vi "read inputs from fpga.vi"(7 "FPGA ref":T6, 8 "error in":errorcluster, 9 "diagnostics":T4[](array[typedef]), 10 "inputs":T1[](array[typedef]), 11 "data table in in":T7) -> (0 "error out":errorcluster, 1 "diagnostics out":T4[](array[typedef]), 2 "inputs out":T1[](array[typedef]), 3 "data table out":T7)   [LabVIEW 2013, in "Profibus Module runtime.lvclass"]
uses:
  Profibus Module runtime.lvclass
  <vilib>/NI/Tag Bus/table/data table.ctl
  profibus diagnostics reporting.ctl
  configuration/error throw specification.ctl
  profibus slave configuration.ctl
  profibus mapping configuration.ctl
  <vilib>/NI/Tag Bus/tag/Data Type.ctl
  dynamic profibus/fpga reference.ctl
  <vilib>/NI/Tag Bus/table/data polymorphs/write one/write Array of U8.vi
  dynamic profibus/dynamic profibus.lvlib
  <vilib>/NI/Tag Bus/table/data table.lvlib
  configuration/Profibus Module configuration.lvclass
  <vilib>/NI/Tag Bus/tag/tag descriptor.lvclass
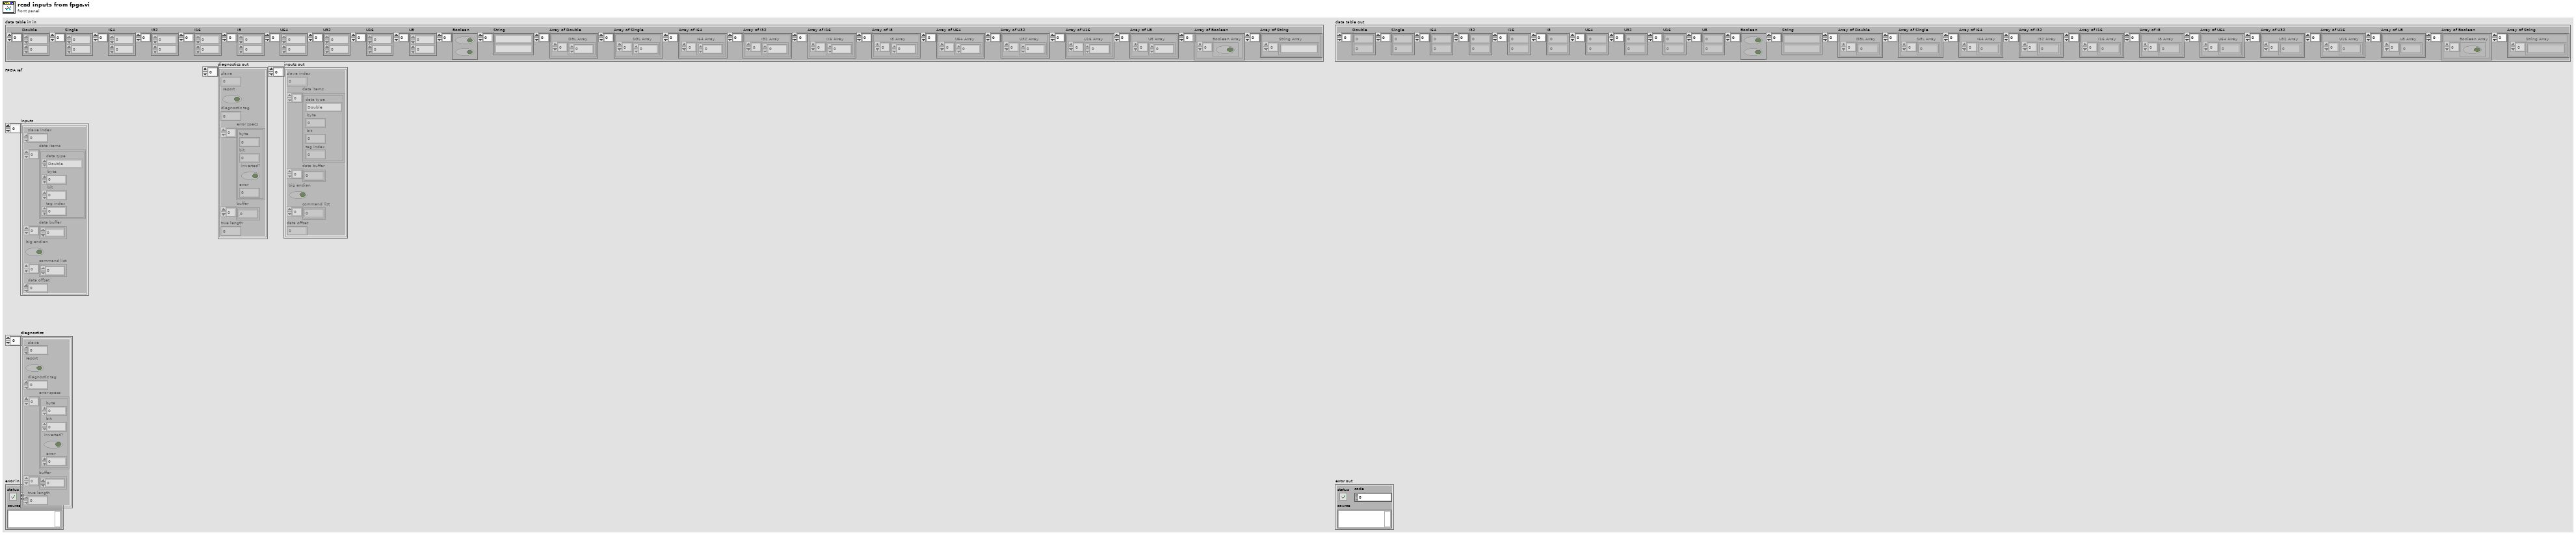
[diagram p1: front panel]
types:
  T1 = typedef "Profibus Module runtime.lvclass/profibus slave configuration.ctl" = cluster{"slave index":i8, "data items":T2[], "data buffer":u8[], "big endian":bool, "command list":u32[], "data offset":u8}
  T2 = typedef "Profibus Module runtime.lvclass/profibus mapping configuration.ctl" = cluster{"data type":T3, " byte":i32, " bit":i32, "tag index":i32}
  T3 = typedef "tag bus.lvlib/tag descriptor.lvclass/Data Type.ctl" = enum16{"Double", "Single", "I64", "I32", "I16", "I8", "U64", "U32", "U16", "U8", "Boolean", "String", "Array of Double", "Array of Single", "Array of I64", "Array of I32", "Array of I16", "Array of I8", "Array of U64", "Array of U32", "Array of U16", "Array of U8", "Array of Boolean", "Array of String"}
  T4 = typedef "Profibus Module runtime.lvclass/profibus diagnostics reporting.ctl" = cluster{"slave":i8, "report":bool, "diagnostic tag":i32, "error specs":T5[], "buffer":u8[], "true length":u8}
  T5 = typedef "Profibus Module configuration.lvclass/error throw specification.ctl" = cluster{"byte":i32, "bit":i32, "inverted?":bool, "error":i32}
  T6 = typedef "dynamic profibus.lvlib/fpga reference.ctl" = refnum<k20>
  T7 = typedef "tag bus.lvlib/data table.lvlib/data table.ctl" = cluster{"Double":dbl[], "Single":sgl[], "I64":i64[], "I32":i32[], "I16":i16[], "I8":i8[], "U64":u64[], "U32":u32[], "U16":u16[], "U8":u8[], "Boolean":bool[], "String":string[], "Array of Double":cluster{"DBL Array":dbl[]}[], "Array of Single":cluster{"SGL Array":sgl[]}[], "Array of I64":cluster{"I64 Array":i64[]}[], "Array of I32":cluster{"I32 Array":i32[]}[], "Array of I16":cluster{"I16 Array":i16[]}[], "Array of I8":cluster{"I8 Array":i8[]}[], "Array of U64":cluster{"U64 Array":u64[]}[], "Array of U32":cluster{"U32 Array":u32[]}[], "Array of U16":cluster{"U16 Array":u16[]}[], "Array of U8":cluster{"U8 Array":u8[]}[], "Array of Boolean":cluster{"Boolean Array":bool[]}[], "Array of String":cluster{"String Array":string[]}[]}
  T8 = typedef "dynamic profibus.lvlib/profibus master transmit header.ctl" = enum8{"Error", "Input", "Diagnostic", "input size", "output size", "many inputs"}
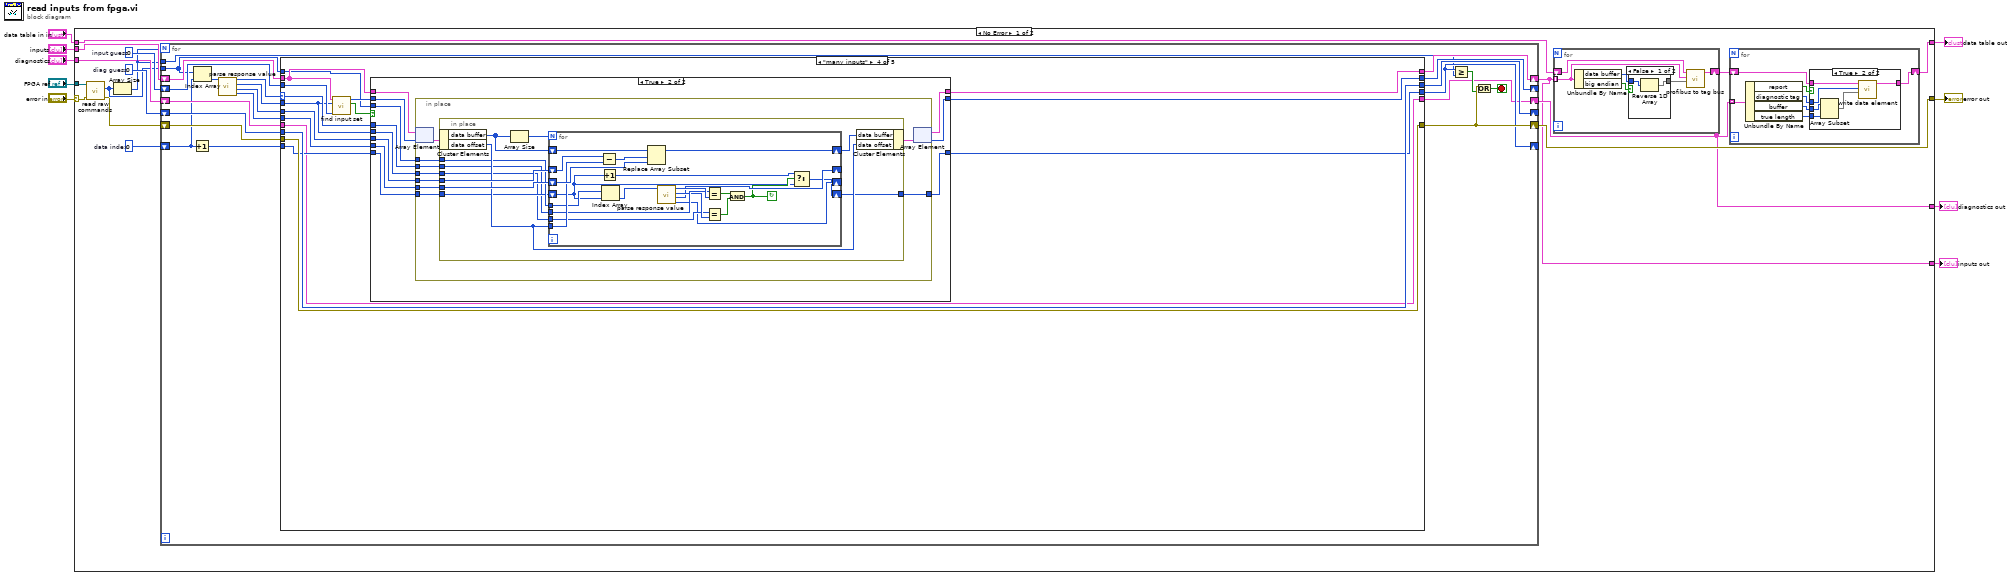
[diagram p0: block diagram]
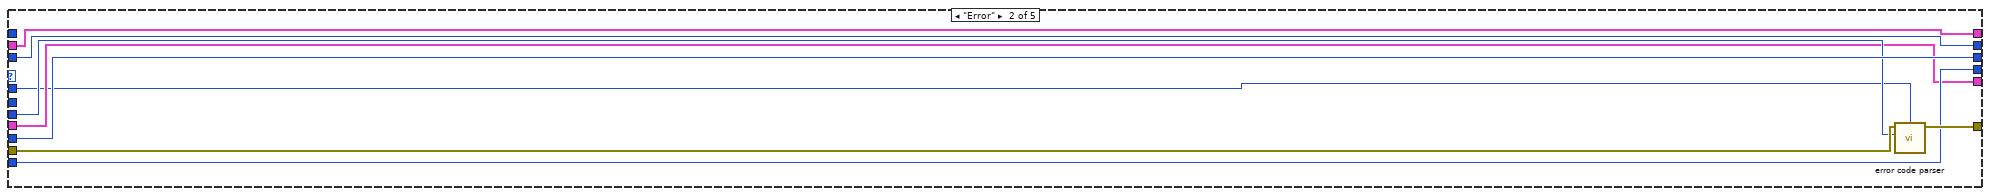
[diagram p4: hidden frame]
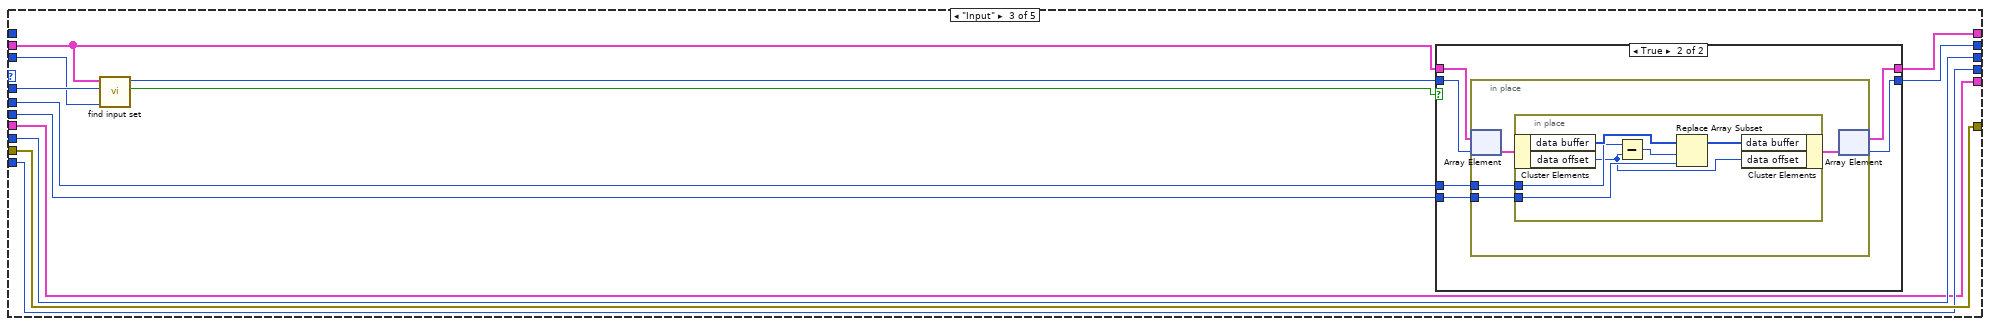
[diagram p5: hidden frame]
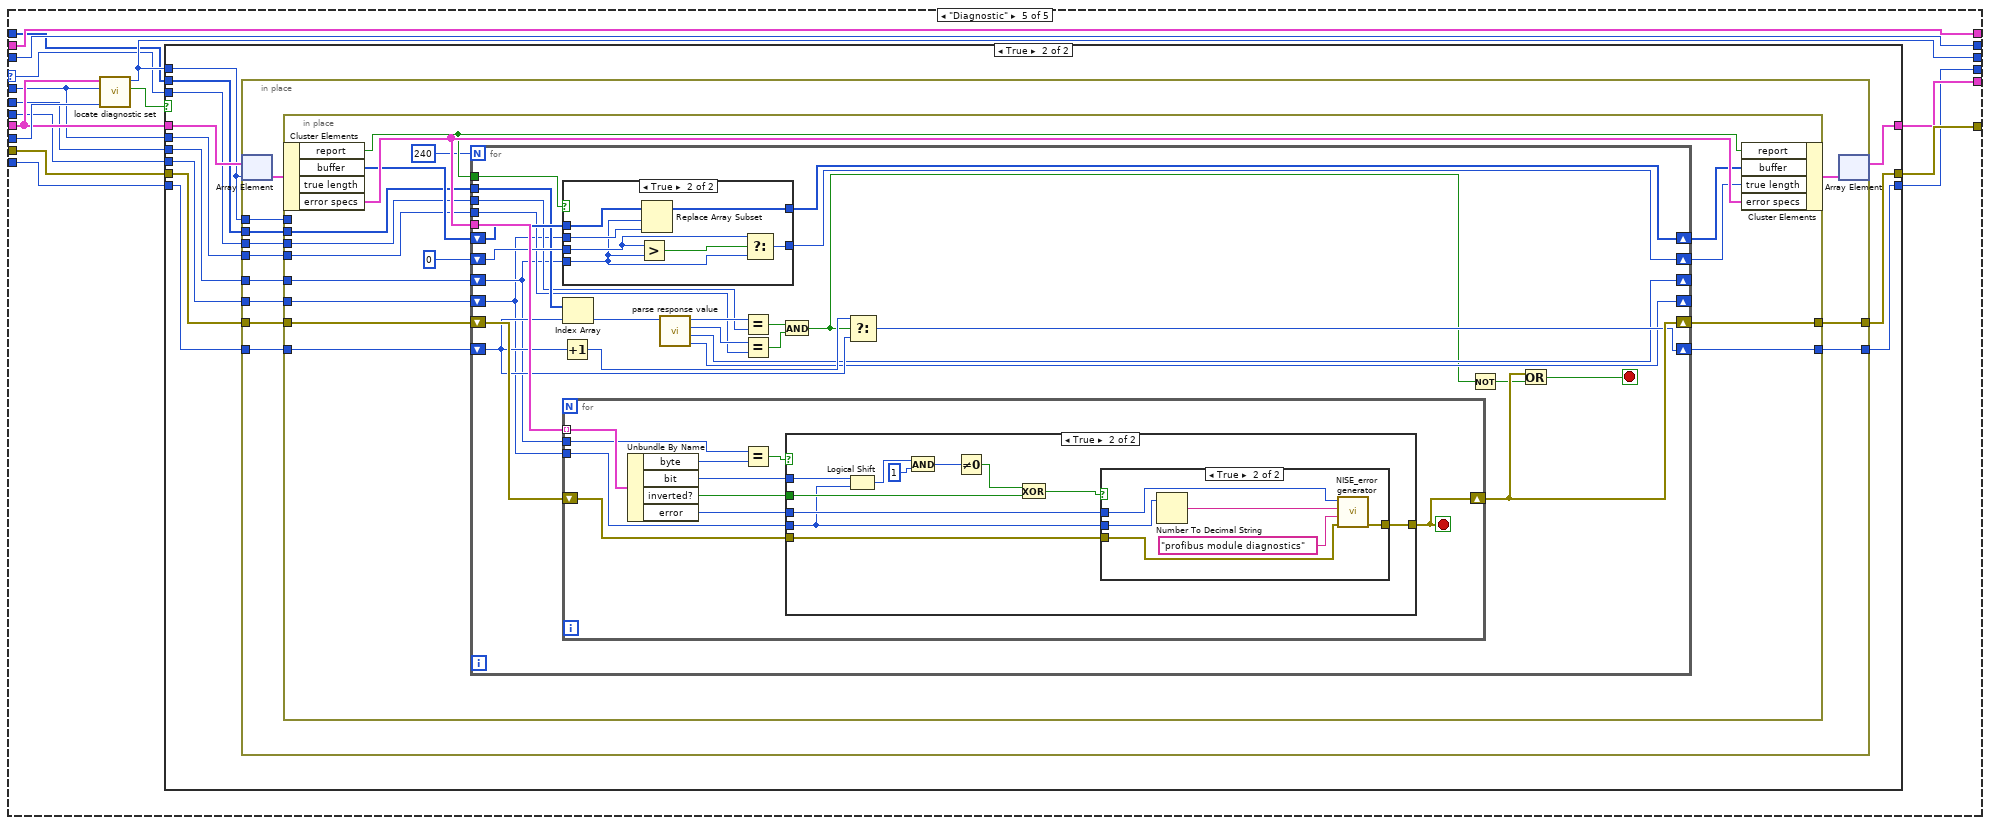
[diagram p8: hidden frame]
diagram:
  n1 = case shown="No Error" "error in" {
    selector: "error in" -> [w19 w313]
    tunnel: "inputs" -> [w24 w310]
    tunnel: [w13 w312] -> w9
    tunnel: [w23 w313] -> w8
    tunnel: "FPGA ref" -> [w20 _]
    tunnel: "diagnostics" -> [w25 w311]
    tunnel: "data table in in" -> [w15 w312]
    tunnel: [w12 w311] -> w2
    tunnel: [w11 w310] -> w1
    frame No Error {
      w18 = 0  # data index
      w21 = 0  # diag guess
      w22 = 0  # input guess
      n2 = call "read raw commands.vi"("error in"=w19, "profibus reference"=w20) -> ("error out"=w10:errorcluster, "Data"=w17:u32[])  [unwired: 7 in, 1 out]
      n3 = Array Size(array=w17) -> (size(s)=w16:i32)
      n4 = for {
        N: w16 -> [_]
        shift-right: [w59] -> w11
        shift-left: w24 -> [w60]
        shift-right: [w57] -> w23
        shift-left: w10 -> [w61]
        shift-right: [w55] -> _
        shift-left: w22 -> [w56]
        shift-right: [w53] -> _
        shift-left: w21 -> [w54]
        tunnel: w17 -> [w45]
        shift-right: [w43] -> _
        shift-left: w18 -> [w48]
        tunnel: w16 -> [w42]
        shift-right: [w40] -> w12
        shift-left: w25 -> [w58]
        stop <- w44 stop-if-true
        n5 = Increment(x=w48) -> (x+1=w47:i32)
        n6 = Index Array(array=w45, index=w48) -> (element=w46:u32)
        n7 = call "parse response value.vi"("Element"=w46) -> ("data"=w49:u8, "index"=w50:u8, "device"=w51:u8, "header"=w52:T8)  [unwired: 7 in]
        n8 = case shown="\"many inputs\"" w52 {
          selector: w52 -> [_ _ _ w110 w181]
          tunnel: w61 -> [w66 w72 w89 w123 w189]
          tunnel: [w66 w73 w89 w123 w190] -> w57
          tunnel: w51 -> [_ w68 w88 w109 w180]
          tunnel: w49 -> [_ w71 w80 w115 w178]
          tunnel: w60 -> [w67 w76 w85 w120 w193]
          tunnel: [w67 w76 w84 w119 w193] -> w59
          tunnel: w50 -> [_ _ w81 w116 w179]
          tunnel: w58 -> [w62 w69 w77 w108 w187]
          tunnel: w56 -> [w65 w75 w87 w122 w192]
          tunnel: [w65 w75 w82 w117 w192] -> w55
          tunnel: w54 -> [w64 w74 w79 w114 w191]
          tunnel: [w64 w74 w79 w114 w186] -> w53
          tunnel: w47 -> [w63 w70 w78 w111 w183]
          tunnel: [w63 w70 w78 w112 w184] -> w43
          tunnel: w45 -> [_ _ _ w113 w182]
          tunnel: [w62 w69 w77 w108 w185] -> w40
          frame "input size", "output size" {
          }
          frame "Error" {
            n9 = call "error code parser.vi"("device"=w68, "Error"=w72, "Status"=w71) -> ("Error out"=w73:errorcluster)  [unwired: 6 in]
          }
          frame "Input" {
            n10 = call "find input set.vi"("input guess in"=w87, "device"=w88, "inputs"=w85) -> ("found?"=w86:bool, "index out"=w83:i32)  [unwired: 7 in]
            n11 = case shown="True" w86 {
              tunnel: w85 -> [w91 w97]
              tunnel: [w91 w95] -> w84
              tunnel: w83 -> [w90 w96]
              tunnel: [w90 w94] -> w82
              tunnel: w81 -> [_ w93]
              tunnel: w80 -> [_ w92]
              frame False {
              }
              frame True {
                n12 = in-place {
                  in-place-border: w93 -> [w99]
                  in-place-border: w92 -> [w98]
                  n13 = in-place-array #1(w97, w96) -> (w101:T1)
                  n14 = in-place {
                    in-place-border: w99 -> [w104]
                    in-place-border: w98 -> [w105]
                    n15 = in-place-cluster #2(w101) -> ("data buffer"=w107:u8[], "data offset"=w102:u8)
                    n16 = Subtract(x=w104, y=w102) -> (x-y=w103:u8)
                    n17 = Replace Array Subset(array=w107, new element=w105, index=w103) -> (w106:u8[])
                    n18 = in-place-cluster #2("data buffer"=w106, "data offset"=w102) -> (w100:T1)
                  }
                  n19 = in-place-array #1(w100) -> (w95:T1[], w94:i32)
                }
              }
            }
          }
          frame "many inputs" {
            n20 = call "find input set.vi"("input guess in"=w122, "device"=w109, "inputs"=w120) -> ("found?"=w121:bool, "index out"=w118:i32)  [unwired: 7 in]
            n21 = case shown="True" w121 {
              tunnel: w120 -> [w126 w137]
              tunnel: [w126 w135] -> w119
              tunnel: w118 -> [w125 w136]
              tunnel: [w125 w134] -> w117
              tunnel: w116 -> [_ w133]
              tunnel: w115 -> [_ w132]
              tunnel: w113 -> [_ w131]
              tunnel: [w124 w127] -> w112
              tunnel: w111 -> [w124 w130]
              tunnel: w110 -> [_ w129]
              tunnel: w109 -> [_ w128]
              frame False {
              }
              frame True {
                n22 = in-place {
                  in-place-border: w133 -> [w144]
                  in-place-border: w132 -> [w143]
                  in-place-border: w131 -> [w142]
                  in-place-border: w130 -> [w141]
                  in-place-border: w129 -> [w140]
                  in-place-border: w128 -> [w139]
                  in-place-border: [w138] -> w127
                  n23 = in-place-array #3(w137, w136) -> (w146:T1)
                  n24 = in-place {
                    in-place-border: w144 -> [w155]
                    in-place-border: w143 -> [w156]
                    in-place-border: w142 -> [w153]
                    in-place-border: w141 -> [w152]
                    in-place-border: w140 -> [w151]
                    in-place-border: w139 -> [w150]
                    in-place-border: [w149] -> w138
                    n25 = in-place-cluster #4(w146) -> ("data buffer"=w148:u8[], "data offset"=w154:u8)
                    n26 = Array Size(array=w148) -> (size(s)=w147:i32)
                    n27 = for {
                      N: w147 -> [_]
                      tunnel: w154 -> [w172]
                      shift-right: [w176] -> w157
                      shift-left: w148 -> [w177]
                      tunnel: w153 -> [w171]
                      shift-right: [w158] -> w149
                      shift-left: w152 -> [w159]
                      tunnel: w151 -> [w168]
                      tunnel: w150 -> [w166]
                      shift-right: [w165] -> _
                      shift-left: w155 -> [w174]
                      shift-right: [w164] -> _
                      shift-left: w156 -> [w175]
                      stop <- w161 continue-if-true
                      n28 = Subtract(x=w174, y=w172) -> (x-y=w173:u8)
                      n29 = Increment(x=w159) -> (x+1=w160:i32)
                      n30 = Index Array(array=w171, index=w159) -> (element=w170:u32)
                      n31 = Replace Array Subset(array=w177, new element=w175, index=w173) -> (w176:u8[])
                      n32 = call "parse response value.vi"("Element"=w170) -> ("data"=w164:u8, "index"=w165:u8, "device"=w167:u8, "header"=w169:T8)  [unwired: 7 in]
                      n33 = Equal?(x=w168, y=w169) -> (x = y?=w162:bool)
                      n34 = Equal?(x=w166, y=w167) -> (x = y?=w163:bool)
                      n35 = And(x=w162, y=w163) -> (x .and. y?=w161:bool)
                      n36 = Select(t=w160, s=w161, f=w159) -> (s? t:f=w158:i32)
                    }
                    n37 = in-place-cluster #4("data buffer"=w157, "data offset"=w154) -> (w145:T1)
                  }
                  n38 = in-place-array #3(w145) -> (w135:T1[], w134:i32)
                }
              }
            }
          }
          frame "Diagnostic" {
            n39 = call "locate diagnostic set.vi"("guess index"=w191, "device"=w180, "diagnostics"=w187) -> ("found?"=w188:bool, "index"=w186:i32)  [unwired: 7 in]
            n40 = case shown="True" w188 {
              tunnel: [w196 w207] -> w190
              tunnel: w189 -> [w196 w208]
              tunnel: w187 -> [w195 w206]
              tunnel: w186 -> [_ w205]
              tunnel: [w195 w204] -> w185
              tunnel: [w194 w202] -> w184
              tunnel: w183 -> [w194 w203]
              tunnel: w182 -> [_ w201]
              tunnel: w181 -> [_ w200]
              tunnel: w180 -> [_ w199]
              tunnel: w179 -> [_ w198]
              tunnel: w178 -> [_ w197]
              frame False {
              }
              frame True {
                n41 = in-place {
                  in-place-border: w205 -> [w220]
                  in-place-border: w208 -> [w219]
                  in-place-border: [w218] -> w207
                  in-place-border: w203 -> [w215]
                  in-place-border: [w214] -> w202
                  in-place-border: w201 -> [w213]
                  in-place-border: w200 -> [w212]
                  in-place-border: w199 -> [w211]
                  in-place-border: w198 -> [w210]
                  in-place-border: w197 -> [w209]
                  n42 = in-place-array #5(w206, w205) -> (w217:T4)
                  n43 = in-place {
                    in-place-border: w220 -> [_]
                    in-place-border: w219 -> [w236]
                    in-place-border: [w235] -> w218
                    in-place-border: w215 -> [w229]
                    in-place-border: [w228] -> w214
                    in-place-border: w213 -> [w227]
                    in-place-border: w212 -> [w226]
                    in-place-border: w211 -> [w225]
                    in-place-border: w210 -> [w224]
                    in-place-border: w209 -> [w223]
                    n44 = in-place-cluster #6(w217) -> ("report"=w231:bool, "buffer"=w233:u8[], "error specs"=w234:T5[])  [unwired: 1 out]
                    n45 = for {
                      N: 240 -> [_]
                      tunnel: w234 -> [w261]
                      tunnel: w231 -> [w258]
                      shift-right: [w257] -> w230
                      shift-left: u8 0 ("true length") -> [w256]
                      shift-right: [w259] -> w232
                      shift-left: w233 -> [w260]
                      shift-right: [w251] -> w228
                      shift-left: w229 -> [w246]
                      shift-right: [w255] -> w235
                      shift-left: w236 -> [w262]
                      tunnel: w227 -> [w254]
                      tunnel: w226 -> [w245]
                      tunnel: w225 -> [w244]
                      shift-right: [w243] -> _
                      shift-left: w224 -> [w241]
                      shift-right: [w242] -> _
                      shift-left: w223 -> [w240]
                      stop <- w239 stop-if-true
                      n46 = Increment(x=w246) -> (x+1=w252:i32)
                      n47 = case shown="True" w258 {
                        tunnel: w260 -> [w293 w300]
                        tunnel: [w293 w298] -> w259
                        tunnel: [w292 w294] -> w257
                        tunnel: w256 -> [w292 w296]
                        tunnel: w241 -> [_ w295]
                        tunnel: w240 -> [_ w299]
                        frame False {
                        }
                        frame True {
                          n48 = Greater?(x=w296, y=w295) -> (0:w297:bool)
                          n49 = Replace Array Subset(array=w300, new element=w299, index=w295) -> (w298:u8[])
                          n50 = Select(t=w296, s=w297, f=w295) -> (s? t:f=w294:u8)
                        }
                      }
                      n51 = Index Array(array=w254, index=w246) -> (element=w253:u32)
                      n52 = for {
                        tunnel: w261 -> [w272] mode=indexing
                        shift-right: [w267] -> w255
                        shift-left: w262 -> [w268]
                        tunnel: w241 -> [w270]
                        tunnel: w240 -> [w264]
                        stop <- w267 stop-if-true
                        n53 = Unbundle By Name(w272) -> ("byte"=w271:i32, "bit"=w266:i32, "inverted?"=w265:bool, "error"=w263:i32)
                        n54 = Equal?(x=w270, y=w271) -> (x = y?=w269:bool)
                        n55 = case shown="True" w269 {
                          tunnel: [w273 w276] -> w267
                          tunnel: w268 -> [w273 w277]
                          tunnel: w266 -> [_ w280]
                          tunnel: w265 -> [_ w279]
                          tunnel: w264 -> [_ w274]
                          tunnel: w263 -> [_ w275]
                          frame False {
                          }
                          frame True {
                            n56 = Logical Shift(y=w280, x=w274) -> (x << y=w284:u8)
                            n57 = And(x=w284, y=u8 1) -> (x .and. y?=w282:u8)
                            n58 = Not Equal To 0?(x=w282) -> (x != 0?=w281:bool)
                            n59 = Exclusive Or(1:w279, 2:w281) -> (0:w278:bool)
                            n60 = case shown="True" w278 {
                              tunnel: w277 -> [w285 w287]
                              tunnel: [w285 w286] -> w276
                              tunnel: w275 -> [_ w289]
                              tunnel: w274 -> [_ w288]
                              frame False {
                              }
                              frame True {
                                n61 = Number To Decimal String(number=w288) -> (decimal integer string=w290:string)  [unwired: 1 in]
                                n62 = call <vilib>:"NISE_error generator.vi"("error in"=w287, "source"="profibus module diagnostics", "append error message"=w290, "error code (0)"=w289) -> ("error out"=w286:errorcluster)  [unwired: 5 in]
                              }
                            }
                          }
                        }
                      }
                      n63 = call "parse response value.vi"("Element"=w253) -> ("data"=w242:u8, "index"=w243:u8, "device"=w249:u8, "header"=w250:T8)  [unwired: 7 in]
                      n64 = Equal?(x=w250, y=w245) -> (x = y?=w247:bool)
                      n65 = Equal?(x=w249, y=w244) -> (x = y?=w248:bool)
                      n66 = And(x=w247, y=w248) -> (x .and. y?=w238:bool)
                      n67 = Select(t=w252, s=w238, f=w246) -> (s? t:f=w251:i32)
                      n68 = Not(x=w238) -> (.not. x?=w237:bool)
                      n69 = Or(x=w255, y=w237) -> (x .or. y?=w239:bool)
                    }
                    n70 = in-place-cluster #6("report"=w231, "buffer"=w232, "true length"=w230, "error specs"=w234) -> (w216:T4)
                  }
                  n71 = in-place-array #5(w216) -> (w204:T4[])  [unwired: 1 out]
                }
              }
            }
          }
        }
        n72 = Greater Or Equal?(x=w43, y=w42) -> (x >= y?=w41:bool)
        n73 = Or(x=w57, y=w41) -> (x .or. y?=w44:bool)
      }
      n74 = for {
        shift-right: [w306] -> w14
        shift-left: w15 -> [w305]
        tunnel: w11 -> [w301] mode=indexing
        n75 = Unbundle By Name(w301) -> ("data buffer"=w302:u8[], "big endian"=w304:bool)
        n76 = case shown="False" w304 {
          tunnel: [w307 w309] -> w303
          tunnel: w302 -> [w308 w309]
          frame False {
            n77 = Reverse 1D Array(array=w308) -> (reversed array=w307:u8[])
          }
          frame True {
          }
        }
        n78 = call "profibus to tag bus.vi"("Data in"=w303, "slave configuration"=w301, "data table in"=w305) -> ("data table out"=w306:T7)  [unwired: 8 in]
      }
      n79 = for {
        shift-right: [w26] -> w13
        shift-left: w14 -> [w27]
        tunnel: w12 -> [w32] mode=indexing
        n80 = Unbundle By Name(w32) -> ("report"=w31:bool, "diagnostic tag"=w30:i32, "buffer"=w29:u8[], "true length"=w28:u8)
        n81 = case shown="True" w31 {
          tunnel: w30 -> [_ w34]
          tunnel: w29 -> [_ w37]
          tunnel: w28 -> [_ w36]
          tunnel: w27 -> [w33 w39]
          tunnel: [w33 w38] -> w26
          frame False {
          }
          frame True {
            n82 = Array Subset(array=w37, length=w36) -> (w35:u8[])  [unwired: 1 in]
            n83 = call-poly <vilib>:"write data element.vi"("value"=w35, "index"=w34, "data table in"=w39) -> ("data table out"=w38:T7)  [unwired: 8 in]
          }
        }
      }
    }
    frame Error {
    }
  }
  "data table out" <- w9
  "error out" <- w8
  "diagnostics out" <- w2
  "inputs out" <- w1
